vi "Checkpoint_Read.vi"(8 "error in (no error)":errorcluster={"status"=FALSE, "code"=0, "source"="\"\""}, 10 "config identity":string, 11 "Checkpoint path":string) -> (0 "error out":errorcluster={"status"=FALSE, "code"=0, "source"="\"\""}, 2 "status ok":bool, 3 "Recovery candidate":string)   [LabVIEW 2026]
doc: "INTENT: Read interrupted-run recovery state. LOGIC: Validate checksum/version/run identity; mark interrupted and require safe-state review."
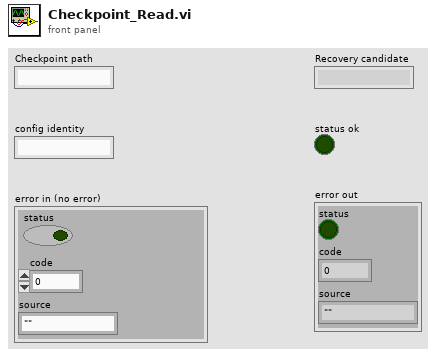
[diagram p1: front panel]
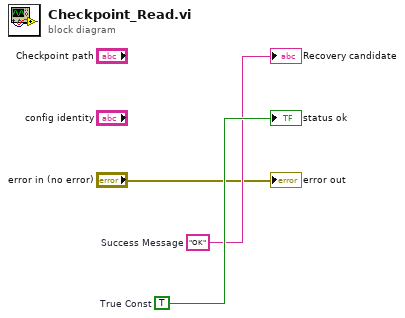
[diagram p0: block diagram]
diagram:
  w3 = TRUE  # True Const
  w2 = "OK"  # Success Message
  "Recovery candidate" <- w2
  "status ok" <- w3
  "error out" <- "error in (no error)"
